vi "Align cRIO Programming Mode.vi"(5 "Password":string, 7 "User Name":string, 8 "error in (no error)":errorcluster, 9 "Local Slots #":u32[](array[numeric]), 10 "FPGAScanInterfaceMode":T1, 11 "Target (localhost)":refnum<k21>="localhost") -> (0 "error out":errorcluster, 2 "Slots Information":T2(array[cluster]) {"Programming Mode" items=["None"=0, "Real-Time CPU"=1, "Real-Time Scan Engine"=2, "LabVIEW FPGA"=4]}, 3 "Slot Programming Mode Supported?":bool)   [LabVIEW 2017, in "Scan Engine Custom Device.lvlib"]
doc: "Based on FPGAScanInterfaceMode input, this VI aligns actual Slot Programming Mode:\n- FPGAScanInterfaceMode = 0 (Use Current), we do nothing. We don't even check current settings (because, it's super slow (SystemConfiguration API)).\n- FPGAScanInterfaceMode = 1 (FPGA) or (Scan mode), we retrieves Product Name and if it's a ni-rio product, checks agains Input list whether it supports the Slot Programming Mode. Then, for detected Slots, we ensure the Slot Programming Mode value is aligned to FPGAScanInterfaceMode and change it if required."
uses:
  Scan Engine Custom Device.lvlib
  Type Defs/FPGAScanInterfaceMode.ctl
  <vilib>/nisyscfg/Filter Mode.ctl
  <vilib>/nisyscfg/Save Changes (Hardware).vi
  <vilib>/nisyscfg/Close (Hardware).vi
  <vilib>/nisyscfg/Close (Filter).vi
  <vilib>/nisyscfg/Close (System).vi
  <vilib>/nisyscfg/nisyscfg.lvlib
  <resource>/objmgr/nicriosae.rc
  <resource>/objmgr/nisysapi.rc
panel:
  # "FPGAScanInterfaceMode:\n0: Use Current\n1: FPGA\n2: Scan mode"
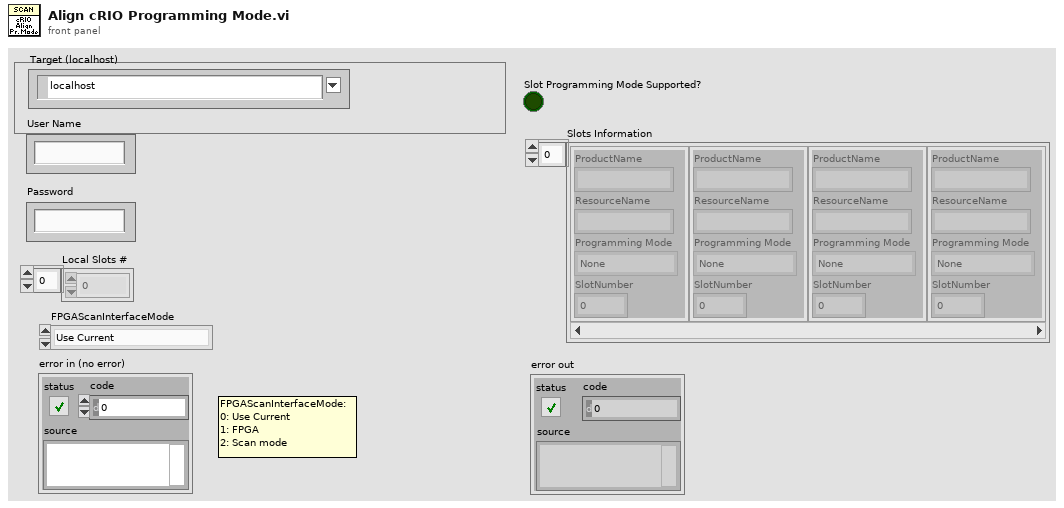
[diagram p1: front panel]
types:
  T1 = typedef "Scan Engine Custom Device.lvlib/FPGAScanInterfaceMode.ctl" = enum16{"Use Current", "FPGA", "Scan mode"}
  T2 = cluster{"ProductName":string, "ResourceName":string, "Programming Mode":u32, "SlotNumber":i32}[]
  T3 = cluster{"ProductName":string, "ResourceName":string, "Programming Mode":u32, "SlotNumber":i32}
  T4 = typedef "nisyscfg.lvlib/Filter Mode.ctl" = i32
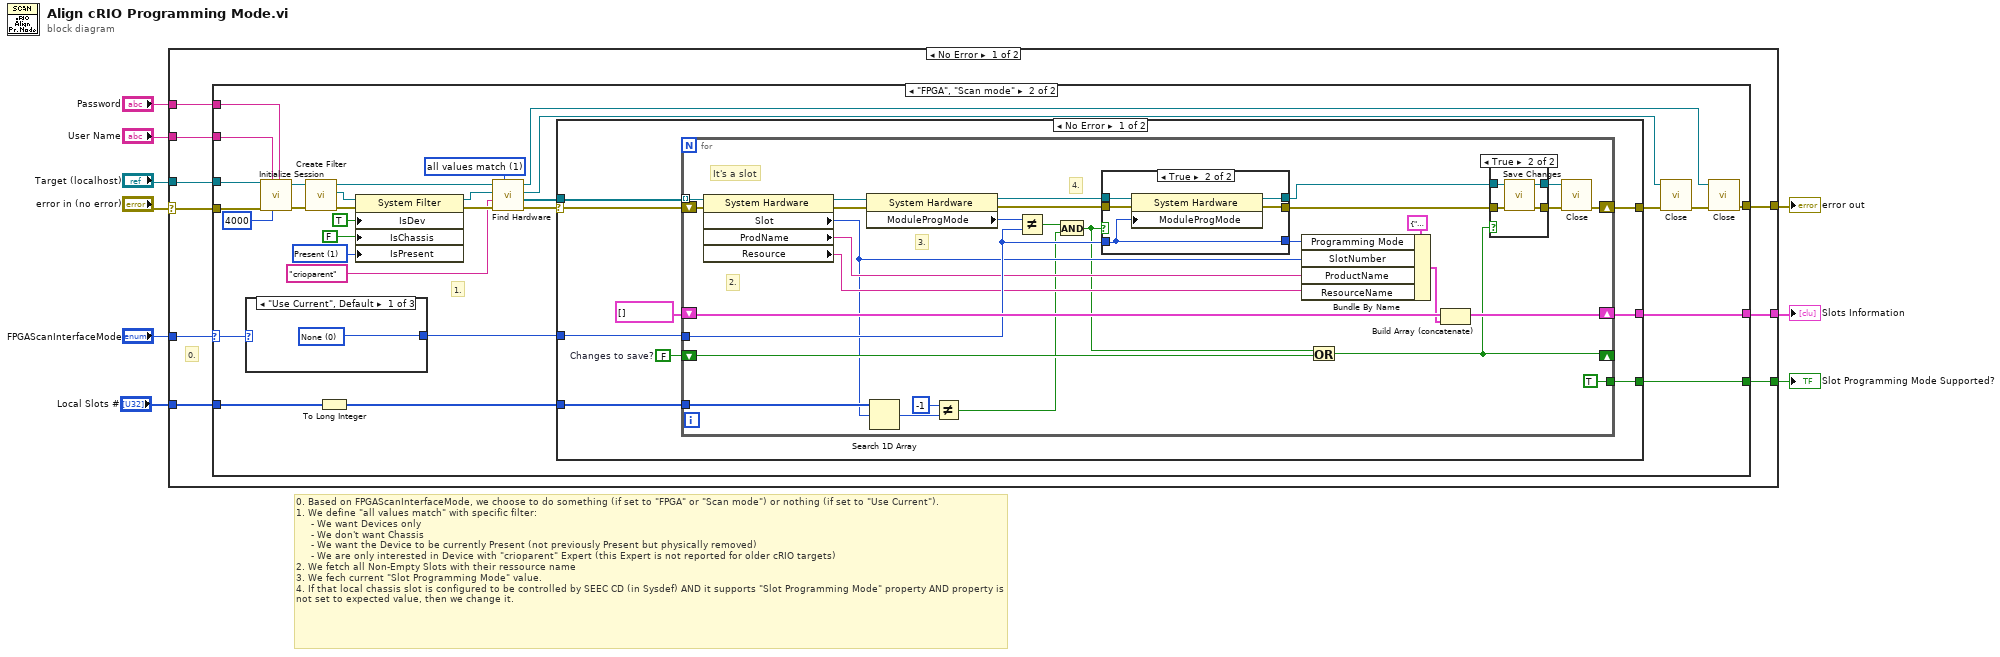
[diagram p0: block diagram]
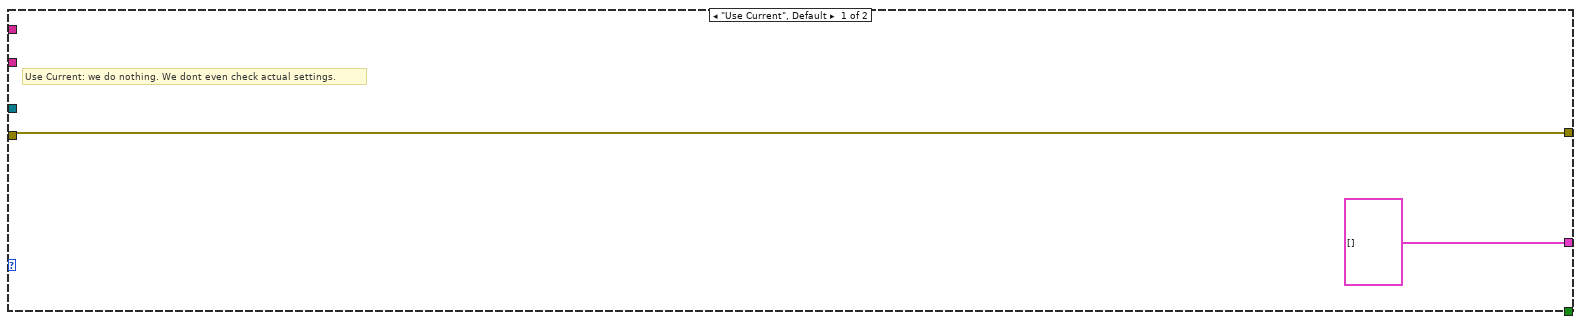
[diagram p2: hidden frame]
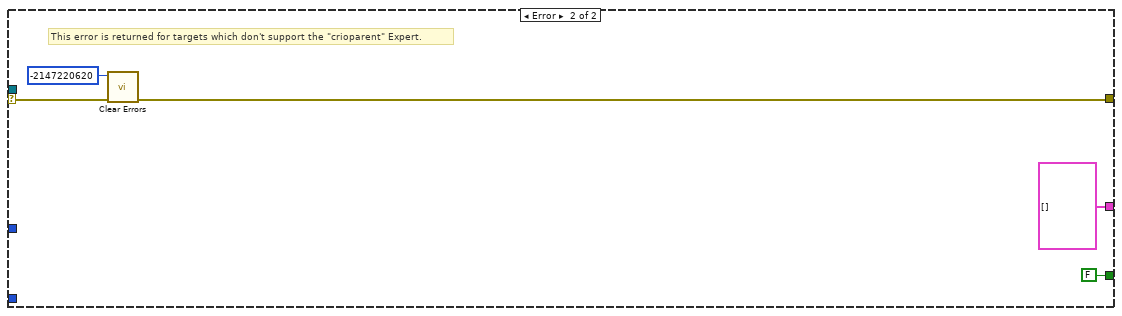
[diagram p5: hidden frame]
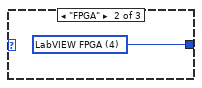
[diagram p6: hidden frame]
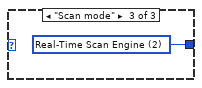
[diagram p7: hidden frame]
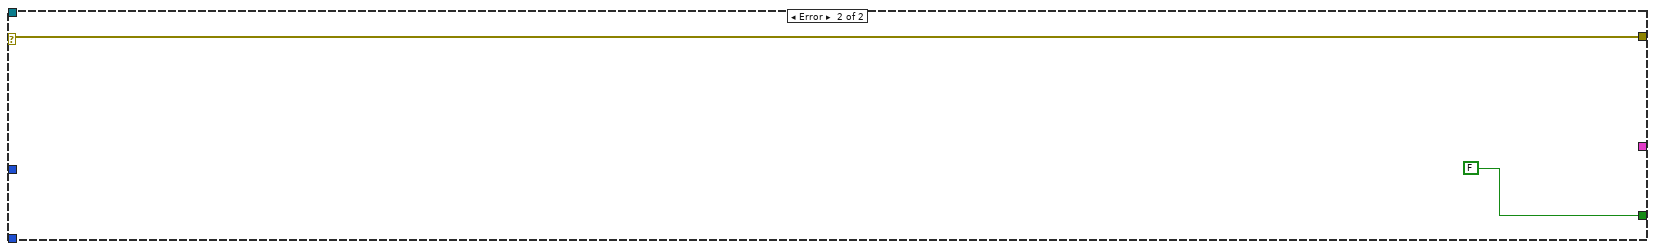
[diagram p8: hidden frame]
diagram:
  # "0. Based on FPGAScanInterfaceMode, we choose to do something (if set to \"FPGA\" or \"Scan mode\") or nothing (if set to \"Use Current\"). \n1. We define \"all values match\" with specific filter:\n     - We want Devices only\n     - We don't want Chassis\n     - We want the Device to be currently Present (not previously Present but physically removed)\n     - We are only interested in Device with \"crioparent\" Expert (this Expert is not reported for older cRIO targets)\n2. We fetch all Non-Empty Slots with their ressource name\n3. We fech current \"Slot Programming Mode\" value.\n4. If that local chassis slot is configured to be controlled by SEEC CD (in Sysdef) AND it supports \"Slot Programming Mode\" property AND property is not set to expected value, then we change it."
  n1 = case shown="No Error" "error in (no error)" {
    selector: "error in (no error)" -> [w13 w113]
    tunnel: "Target (localhost)" -> [w18 _]
    tunnel: "User Name" -> [w17 _]
    tunnel: "Password" -> [w16 _]
    tunnel: [w15 FALSE] -> w6
    tunnel: [w14 w113] -> w5
    tunnel: [w12 _] -> w3
    tunnel: "FPGAScanInterfaceMode" -> [w11 _]
    tunnel: "Local Slots #" -> [w10 _]
    frame No Error {
      # "0."
      n2 = case shown="\"FPGA\", \"Scan mode\"" w11 {
        selector: w11 -> [_ w28]
        tunnel: w18 -> [_ w37]
        tunnel: w17 -> [_ w36]
        tunnel: w16 -> [_ w35]
        tunnel: [_ w32] -> w15
        tunnel: [w20 w31] -> w14
        tunnel: w13 -> [w20 w30]
        tunnel: [T2 [] w29] -> w12
        tunnel: w10 -> [_ w23]
        frame "Use Current", Default {
          # "Use Current: we do nothing. We dont even check actual settings."
        }
        frame "FPGA", "Scan mode" {
          w25 = 1 items=["Initializing"=-2, "Unknown"=-1, "Not Present"=0, "Present"=1] ("Devices & Chassis:Is Present")
          w41 = T4 1 items=["all values match"=1, "any value matches"=2, "values do not match"=3, "all properties exist"=4] ("filter mode (all values match)")
          # "1."
          n3 = case shown="\"Use Current\", Default" w28 {
            tunnel: [w109 w110 w111] -> w27
            frame "Use Current", Default {
              w109 = u32 0 items=["None"=0, "Real-Time CPU"=1, "Real-Time Scan Engine"=2, "LabVIEW FPGA"=4] ("Programming Mode")
            }
            frame "FPGA" {
              w110 = u32 4 items=["None"=0, "Real-Time CPU"=1, "Real-Time Scan Engine"=2, "LabVIEW FPGA"=4] ("Programming Mode")
            }
            frame "Scan mode" {
              w111 = u32 2 items=["None"=0, "Real-Time CPU"=1, "Real-Time Scan Engine"=2, "LabVIEW FPGA"=4] ("Programming Mode")
            }
          }
          n4 = call <vilib>:"Initialize Session.vi"("Password"=w35, "Connect Timeout (4000 ms)"=u32 4000, "User Name"=w36, "error in (no error)"=w30, "Target (localhost)"=w37) -> ("error out"=w43:errorcluster, "Session out"=w46:refnum<k21>)  [unwired: 5 in]
          n5 = call <vilib>:"Create Filter.vi"("error in (no error)"=w43, "Session in"=w46) -> ("error out"=w48:errorcluster, "Filter out"=w47:refnum<k20>, "Session out"=w45:refnum<k21>)  [unwired: 7 in]
          n6 = To Long Integer(number=w23) -> (32bit integer=w22:i32[])
          n7 = property class="System Filter"(reference=w47, error in=w48, "IsDev"=TRUE ("Is Device"), "IsChassis"=FALSE ("Is Chassis"), "IsPresent"=w25) -> (reference out=w42:refnum<k20>, error out=w44:errorcluster)
          n8 = call <vilib>:"Find Hardware.vi"("Filter Mode (all values match)"=w41, "error in (no error)"=w44, "Experts"="crioparent" ("Expert Info:Expert Name"), "Filter in"=w42, "Session in"=w45) -> ("error out"=w21:errorcluster, "Resources out"=w50:refnum<k20>[], "Filter out"=w39:refnum<k20>, "Session out"=w49:refnum<k21>)  [unwired: 3 out]
          n9 = case shown="No Error" w21 {
            selector: w21 -> [w51 w108]
            tunnel: w50 -> [w59 _]
            tunnel: [w58 w106] -> w38
            tunnel: [w57 FALSE] -> w32
            tunnel: [w55 T2 []] -> w29
            tunnel: w27 -> [w54 _]
            tunnel: w22 -> [w52 _]
            frame No Error {
              w53 = FALSE  # Changes to save?
              n10 = for {
                tunnel: w59 -> [w80] mode=indexing
                shift-right: [w89] -> w58
                shift-left: w51 -> [w77]
                shift-right: [w87] -> w55
                shift-left: T2 [] -> [w88]
                tunnel: w54 -> [w86]
                shift-right: [w82] -> _
                shift-left: w53 -> [w85]
                tunnel: w52 -> [w74]
                tunnel: [TRUE] -> w57
                # "4."
                # "3."
                # "2."
                # "It's a slot"
                n11 = property class="System Hardware"(reference=w80, error in=w77) -> (reference out=w79:refnum<k20>, error out=w78:errorcluster, "Slot"=w73:i32, "ProdName"=w76:string, "Resource"=w75:string)
                n12 = property class="System Hardware"(reference=w79, error in=w78) -> (reference out=w70:refnum<k20>, error out=w69:errorcluster, "ModuleProgMode"=w67:u32)
                n13 = Search 1D Array(1D array=w74, element=w73) -> (index of element=w64:i32)  [unwired: 1 in]
                n14 = Not Equal?(x=-1, y=w64) -> (x != y?=w61:bool)
                n15 = Not Equal?(x=w67, y=w86) -> (x != y?=w62:bool)
                n16 = And(x=w62, y=w61) -> (x .and. y?=w60:bool)
                n17 = case shown="True" w60 {
                  tunnel: w70 -> [w98 w103]
                  tunnel: w69 -> [w97 w101]
                  tunnel: [w98 w102] -> w72
                  tunnel: w86 -> [w96 w99]
                  tunnel: [w97 w100] -> w71
                  tunnel: [w96 w99] -> w68
                  frame False {
                    # "Already set with right Pr. mode.\nor absent."
                  }
                  frame True {
                    n18 = property class="System Hardware"(reference=w103, error in=w101, "ModuleProgMode"=w99) -> (reference out=w102:refnum<k20>, error out=w100:errorcluster)
                  }
                }
                n19 = Bundle By Name(cluster=T3 {"ProductName"="", "ResourceName"="", "Programming Mode"=0, "SlotNumber"=0}, "Programming Mode"=w68, "SlotNumber"=w73, "ProductName"=w76, "ResourceName"=w75) -> (w65:T3)
                n20 = Or(x=w60, y=w85) -> (x .or. y?=w82:bool)
                n21 = Build Array (concatenate)(w88, w65) -> (w87:T2)
                n22 = case shown="True" w82 {
                  tunnel: w72 -> [w91 w95]
                  tunnel: w71 -> [w90 w94]
                  tunnel: [w90 w93] -> w84
                  tunnel: [w91 w92] -> w83
                  frame False {
                  }
                  frame True {
                    n23 = call-poly <vilib>:"Save Changes.vi"("error in (no error)"=w94, "Resource in"=w95) -> ("error out"=w93:errorcluster, "Resource out"=w92:refnum<k20>)  [unwired: 6 in, 2 out]
                  }
                }
                n24 = call-poly <vilib>:"Close.vi"("error in (no error)"=w84, "Resource in"=w83) -> ("error out"=w89:errorcluster)  [unwired: 9 in]
              }
            }
            frame Error {
              # "This error is returned for targets which don't support the \"crioparent\" Expert."
              n25 = call <vilib>:"Clear Errors.vi"("error in (no error)"=w108, "specific error code to clear (0: all)"=-2147220620) -> ("error out"=w106:errorcluster)  [unwired: 4 in, 1 out]
            }
          }
          n26 = call-poly <vilib>:"Close.vi"("error in (no error)"=w38, "Filter in"=w39) -> ("error out"=w40:errorcluster)  [unwired: 9 in]
          n27 = call-poly <vilib>:"Close.vi"("error in (no error)"=w40, "Session in"=w49) -> ("error out"=w31:errorcluster)  [unwired: 9 in]
        }
      }
    }
    frame Error {
    }
  }
  "Slot Programming Mode Supported?" <- w6
  "error out" <- w5
  "Slots Information" <- w3
